vi "Read CAN.vi"() -> ()   [LabVIEW 2021]
uses:
  <vilib>/CIF Foundation/CIF CAN RW Core/typedef/CAN Port Configuration.ctl
  <vilib>/CIF Foundation/CIF CAN RW Core/typedef/CAN Mode.ctl
  <vilib>/CIF Foundation/CIF CAN RW Core/typedef/FD Config.ctl
  <vilib>/xnet/xnet.llb/XNET Frame CAN.ctl
  <vilib>/xnet/xnet.llb/XNET Frame Type CAN.ctl
  <vilib>/CIF Foundation/CIF CAN RW Core/typedef/Statistics.ctl
  <vilib>/CIF Foundation/CIF XNET CAN RW/XNET CAN RW.lvclass
  C:/Program Files/National Instruments/LabVIEW 2021/vi.lib/CIF Foundation/CIF CAN RW Core/CAN_RW_CORE.lvclass
  <vilib>/CIF Foundation/CIF CAN RW Core/CAN_RW_CORE.lvclass/CAN_RW_CORE.ctl
  <vilib>/CIF Foundation/CIF PCAP Parse and Build/pcap_Parse_Build_CIF.lvclass/pcap_Parse_Build_CIF.ctl
  <vilib>/CIF Foundation/CIF XNET CAN RW/Utilities/Header Cluster to XNET CAN.vi
  <vilib>/CIF Foundation/CIF PCAP Parse and Build/Parse/Parse Packet Header.vi
  <vilib>/CIF Foundation/CIF PCAP Parse and Build/Parse/Unflatten Socket CAN Header.vi
  <vilib>/CIF Foundation/CIF PCAP Parse and Build/Utilities/Get Data Segment.vi
  <vilib>/CIF Foundation/CIF PCAP Parse and Build/Data Accessors/Read Offset.vi
  <vilib>/CIF Foundation/CIF CAN RW Core/Utilities/Filter Packets.vi
  <vilib>/CIF Foundation/CIF CAN RW Core/Accessors/Read pcap class.vi
  <vilib>/CIF Foundation/CIF CAN RW Core/Accessors/Write pcap class.vi
  <vilib>/CIF Foundation/CIF PCAP Parse and Build/Data Accessors/Write Offset.vi
  <vilib>/dlg_ctls.llb/Space Constant.vi
  <vilib>/CIF Foundation/CIF Utilities/Time/System Time/TAI Time to LabVIEW Time.vi
  <vilib>/CIF Foundation/CIF PCAP Parse and Build/Parse/Unflatten Packet Header.vi
  <vilib>/CIF Foundation/CIF Utilities/DataTypes/Flatten Unflatten/Unflatten U32.vi
  <vilib>/CIF Foundation/CIF PCAP Parse and Build/Utilities/Add Error.vi
  <vilib>/CIF Foundation/CIF Utilities/Errors/Append Error Location.vi
  <vilib>/CIF Foundation/CIF PCAP Parse and Build/pcap_Parse_Build_CIF.lvclass
  <vilib>/CIF Foundation/CIF CAN RW Core/CAN_RW_CORE.lvclass
panel:
  in  "stop":bool
  out "Plugin Status":string[][](table)
  out "Statistcs":T1
  out "CAN":T2[](array[typedef]) {"payload" format="%x"; "timestamp" format="%<%.7X\n%x>T"; "type" items=["CAN Data"=0, "CAN Remote"=1, "CAN Bus Error"=2, "CAN 2.0 Data"=8, "CAN FD Data"=16, "CAN FD+BRS Data"=24, "J1939 Data"=192, "Delay"=224, "Log Trigger"=225, "Start Trigger"=226]; "identifier" format="%x"}
  out "error out":errorcluster
  in  "Port Configuration":T4={"Mode"=enum."CAN FD", "Baud Rate"=500000, "Temination On"=TRUE, "Subordinate"=FALSE, "Echo TX"=FALSE, "FD Config"={"FD Baud Rate"=2000000, "ISO Mode"=TRUE, "BRS Enabled"=TRUE}} {"FD Config"."FD Baud Rate" format="%.0p"; "Baud Rate" format="%.0p"}
  in  "RX Initerface":string="CAN2"
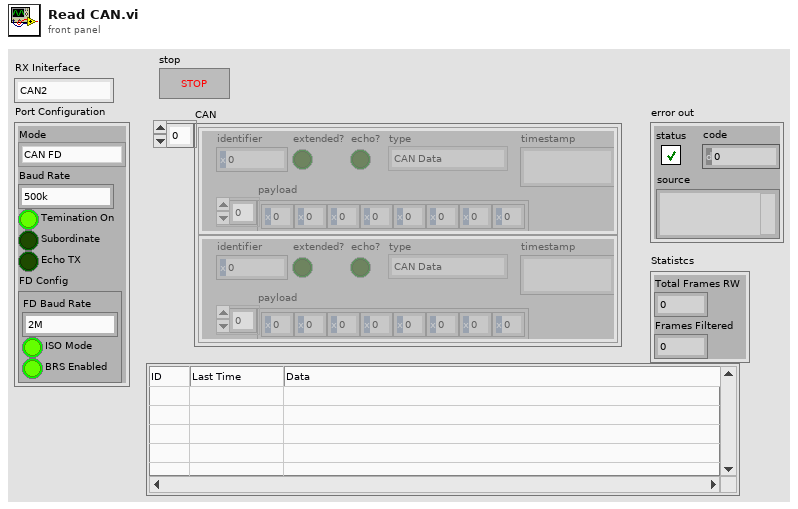
[diagram p1: front panel]
types:
  T1 = typedef "CAN_RW_CORE.lvclass/Statistics.ctl" = cluster{"Total Frames RW":u32, "Frames Filtered ":u32}
  T2 = typedef "XNET Frame CAN.ctl" = cluster{"timestamp":timestamp, "payload":u8[], "identifier":u32, "type":T3, "extended?":bool, "echo?":bool}
  T3 = typedef "XNET Frame Type CAN.ctl" = u8
  T4 = typedef "CAN_RW_CORE.lvclass/CAN Port Configuration.ctl" = cluster{"Mode":T5, "Baud Rate":u64, "Temination On":bool, "Subordinate":bool, "Echo TX":bool, "FD Config":T6}
  T5 = typedef "CAN_RW_CORE.lvclass/CAN Mode.ctl" = enum16{"CAN 2.0", "CAN FD"}
  T6 = typedef "CAN_RW_CORE.lvclass/FD Config.ctl" = cluster{"FD Baud Rate":u64, "ISO Mode":bool, "BRS Enabled":bool}
  T7 = typedef "XNET CAN RW.lvclass/CAN Return Map.ctl" = map{u32, T2}
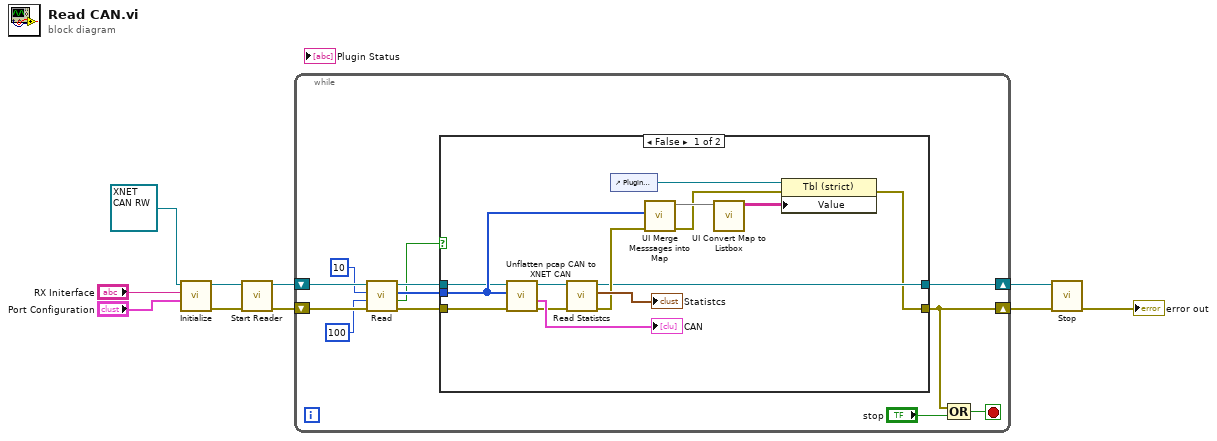
[diagram p0: block diagram]
diagram:
  n1 = call <vilib>:"Initialize.vi"("Port Configuration"="Port Configuration", "Interface"="RX Initerface", "XNET_CAN_RW in"=refnum<class "XNET CAN RW.lvclass"> refnum ("CAN_Logic in")) -> ("error out"=w8:errorcluster, "XNET_CAN_RW out"=w9:refnum<class "XNET CAN RW.lvclass">)  [unwired: 7 in]
  n2 = call-dynamic "Start Reader.vi"("error in (no error)"=w8, "XNET_CAN_RW in"=w9) -> ("error out"=w4:errorcluster, "XNET_CAN_RW out"=w5:refnum<class "XNET CAN RW.lvclass">)  [unwired: 8 in]
  n3 = while {
    shift-right: [w17] -> w3
    shift-left: w5 -> [w22]
    shift-right: [w13] -> w2
    shift-left: w4 -> [w20]
    stop <- w11 stop-if-true
    n4 = call-dynamic "Read.vi"("error in (no error)"=w20, "timeout (ms)"=100, "number to read"=10, "XNET_CAN_RW in"=w22) -> ("error out"=w18:errorcluster, "Timeout"=w14:bool, "pcap CAN Data"=w21:u8[], "XNET_CAN_RW out"=w19:refnum<class "XNET CAN RW.lvclass">)  [unwired: 3 in, 1 out]
    n5 = case shown="False" w14 {
      tunnel: w21 -> [w31 _]
      tunnel: w19 -> [w27 w38]
      tunnel: w18 -> [w26 w37]
      tunnel: [w25 w38] -> w17
      tunnel: [w24 w37] -> w13
      frame False {
        n6 = call <vilib>:"Unflatten pcap CAN to XNET CAN.vi"("error in (no error)"=w26, "pcap CAN DATA in"=w31, "XNET_CAN_RW in"=w27) -> ("error out"=w29:errorcluster, "XNET CAN Data"=→"CAN":T2[], "XNET_CAN_RW out"=w35:refnum<class "XNET CAN RW.lvclass">)  [unwired: 3 in, 3 out]
        n7 = call <vilib>:"Read Statistcs.vi"("error in (no error)"=w29, "CAN_RW_CORE in"=w35) -> ("error out"=w28:errorcluster, "Statistcs"=→"Statistcs":T1, "CAN_RW_CORE out"=w25:refnum<class "XNET CAN RW.lvclass">)  [unwired: 7 in]
        n8 = control-ref of="Plugin Status"() -> (w30:refnum<vi>)
        n9 = call <vilib>:"UI Merge Messsages into Map.vi"("error in (no error)"=w28, "pcap CAN DATA in"=w31) -> ("error out"=w23:errorcluster, "CAN Return MAP out"=w33:T7)  [unwired: 8 in]
        n10 = call <vilib>:"UI Convert Map to Listbox.vi"("CAN Return MAP in"=w33) -> ("CAN Data for Mutli Listbox"=w32:string[][])  [unwired: 10 in]
        n11 = property class="Tbl (strict)"(reference=w30, error in=w23, "Value"=w32) -> (error out=w24:errorcluster)  [unwired: 1 out]
      }
      frame True {
      }
    }
    n12 = Compound Arithmetic op=OR(w13, "stop") -> (w11:bool)
  }
  n13 = call-dynamic "Stop.vi"("error in (no error)"=w2, "XNET_CAN_RW in"=w3) -> ("error out"=→"error out":errorcluster)  [unwired: 8 in, 1 out]
